vi "set HO Uplink Channel.vi"(8 "error in (no error)":errorcluster caption="에러 입력(에러 없음)", 9 "UL Channel Arguments":T2, 10 "UL Channel Info":T1, 11 "LTE 입력":refnum<class "LTE.lvclass">) -> (0 "error out":errorcluster caption="에러 출력", 3 "LTE 출력":refnum<class "LTE.lvclass">)   [LabVIEW 2023, in "ANRITSU Call Box.lvlib" / "LTE.lvclass"]
uses:
  LTE.lvclass
  LTE.lvclass/LTE.ctl
  Type Definition/LTE Uplink Channel Number Target.ctl
  ANRITSU Call Box.lvlib
  Type Definition/LTE Uplink Channel Number Info.ctl
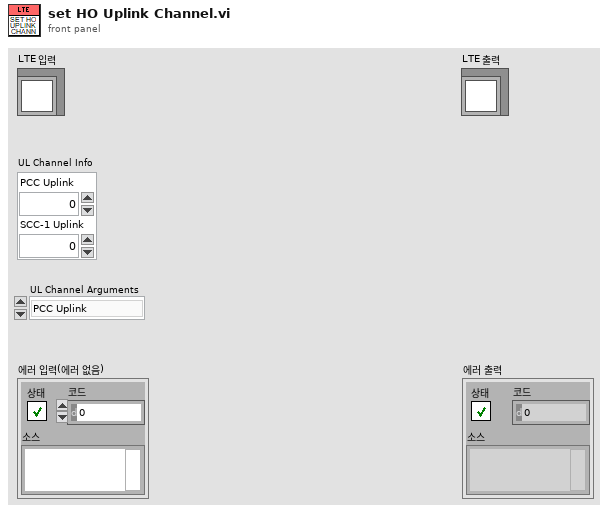
[diagram p1: front panel]
types:
  T1 = typedef "ANRITSU Call Box.lvlib/LTE Uplink Channel Number Info.ctl" = cluster{"PCC Uplink":i32, "SCC-1 Uplink":i32}
  T2 = typedef "ANRITSU Call Box.lvlib/LTE Uplink Channel Number Target.ctl" = enum16{"PCC Uplink", "SCC-1 Uplink", "All"}
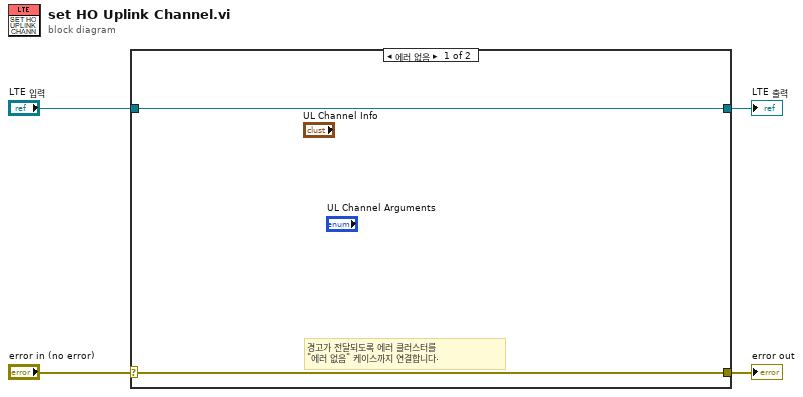
[diagram p0: block diagram]
diagram:
  n1 = case shown="에러 없음" "error in (no error)" {
    selector: "error in (no error)" -> [w5 w8]
    tunnel: [w5 w8] -> w3
    tunnel: [w6 w7] -> w1
    tunnel: "LTE 입력" -> [w6 w7]
    frame No Error {
      # "경고가 전달되도록 에러 클러스터를\n\"에러 없음\" 케이스까지 연결합니다."
    }
    frame Error {
    }
  }
  "error out" <- w3
  "LTE 출력" <- w1
